vi "lvmcp_invokeconfig.vi"() -> ()   [LabVIEW 2015]
panel:
  out "reference out":refnum<vi>
  out "error out":errorcluster
  in  "reference":refnum<vi>
  in  "Allow Alternate Names? (F)":bool
  in  "ID String":string
  in  "Invoke Node Class Name":string
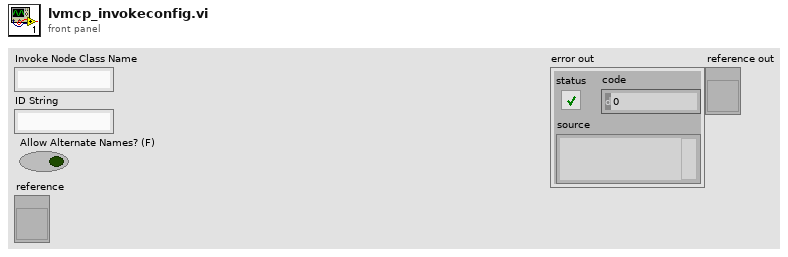
[diagram p1: front panel]
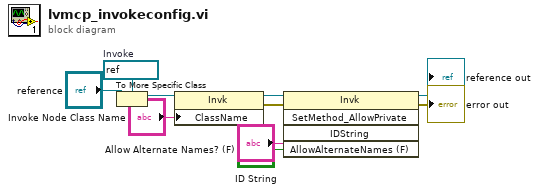
[diagram p0: block diagram]
diagram:
  w10 = refnum<vi> refnum  # Invoke
  n1 = To More Specific Class(target class=w10, reference="reference") -> (specific class reference=w9:refnum<vi>)  [unwired: 1 in, 1 out]
  n2 = property class="Invk"(reference=w9, "ClassName"="Invoke Node Class Name") -> (reference out=w7:refnum<vi>, error out=w6:errorcluster)  [unwired: 1 in]
  n3 = invoke class="Invk" method="SetMethod_AllowPrivate"(reference=w7, error in=w6, "IDString"="ID String", "AllowAlternateNames (F)"="Allow Alternate Names? (F)") -> (reference out=→"reference out":refnum<vi>, error out=→"error out":errorcluster)  [unwired: 1 in, 3 out]
